vi "close.vi"(8 "error in (no error)":errorcluster, 11 "rotationTable in":refnum<class "rotationTable.lvclass">) -> (0 "error out":errorcluster, 3 "rotationTable out":refnum<class "rotationTable.lvclass">)   [LabVIEW 2020, in "rotationTable.lvclass"]
uses:
  rotationTable.lvclass
  rotationTable.lvclass/rotationTable.ctl
  lexitekDriver_client/lexitekDriver_client.lvlib
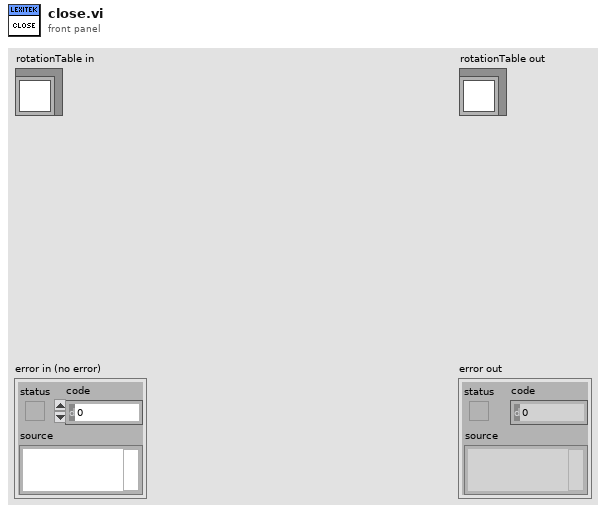
[diagram p1: front panel]
types:
  T1 = typedef "grpc-lvsupport-release.lvlib/grpcId.ctl" = u64
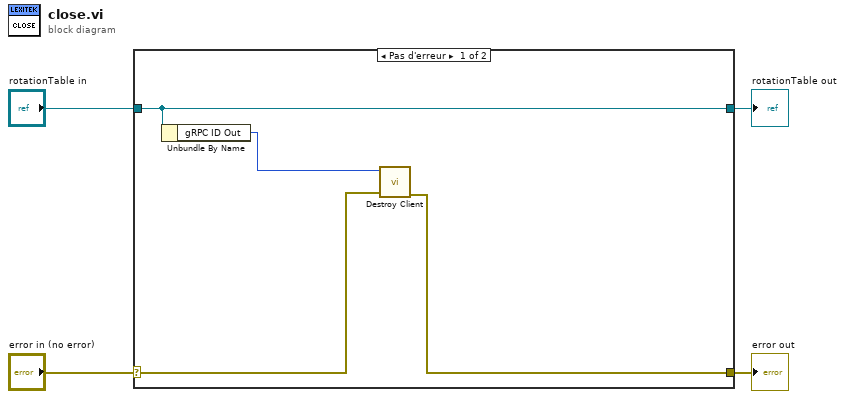
[diagram p0: block diagram]
diagram:
  n1 = case shown="Pas d'erreur" "error in (no error)" {
    selector: "error in (no error)" -> [w6 w10]
    tunnel: [w5 w10] -> w3
    tunnel: [w8 w9] -> w1
    tunnel: "rotationTable in" -> [w8 w9]
    frame No Error {
      n2 = Unbundle By Name(w8) -> ("gRPC ID Out"=w7:T1)
      n3 = call "Destroy Client.vi"("error in"=w6, "gRPC ID"=w7) -> ("error out"=w5:errorcluster)  [unwired: 9 in]
    }
    frame Error {
    }
  }
  "error out" <- w3
  "rotationTable out" <- w1
